vi "RemoteVI Launch Share.vi"(0 "VI":refnum<vi>, 1 "whole network?":bool, 2 "token":string, 3 "view only?":bool, 5 "port":u16=8088, 7 "fps":dbl=20.0, 8 "VI Server":string, 9 "window":u64, 10 "loop VI":path, 11 "error in":errorcluster) -> (4 "URL":string, 15 "error out":errorcluster)   [LabVIEW 2020, in "RemoteVI.lvlib"]
doc: "Starts one share (RemoteVI Start.vi and RemoteVI Start Window.vi call it): makes the access token (the given one or RemoteVI New Token.vi), the link (http://127.0.0.1:<port>/?t=... - or this computer's IP address with whole network?), refuses a port this application instance shares already (error 5001, RemoteVI Share Running.vi), opens a new clone of the reentrant RemoteVI Server Loop.vi, sets its controls and runs it (RemoteVI Launch Server Loop.vi), and waits until it listens (its listener error, e.g. 60; 5002 after 2 s). window not 0 shares that window of any process instead of VI (a window target). loop VI (not empty) runs that VI instead of the Server Loop (RemoteVI Start Landing Page.vi: the landing page)."
uses:
  RemoteVI.lvlib
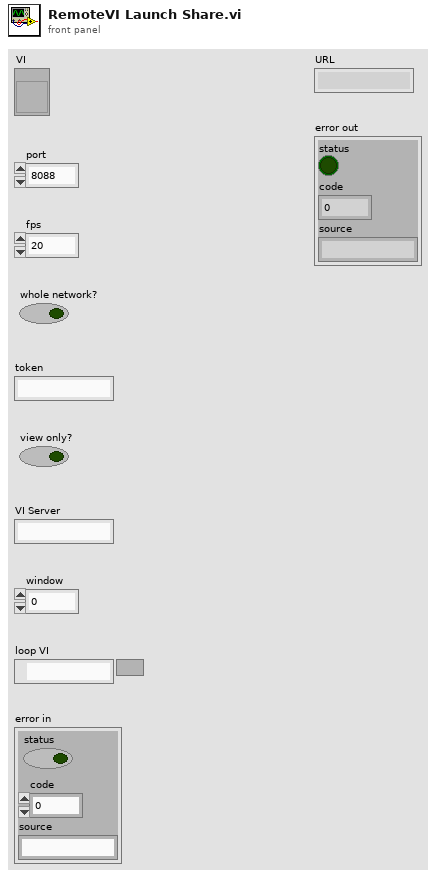
[diagram p1: front panel]
types:
  T1 = cluster{"token":string, "net address":u32, "url":string, "view only":bool, "whole network":bool, "window":u64}
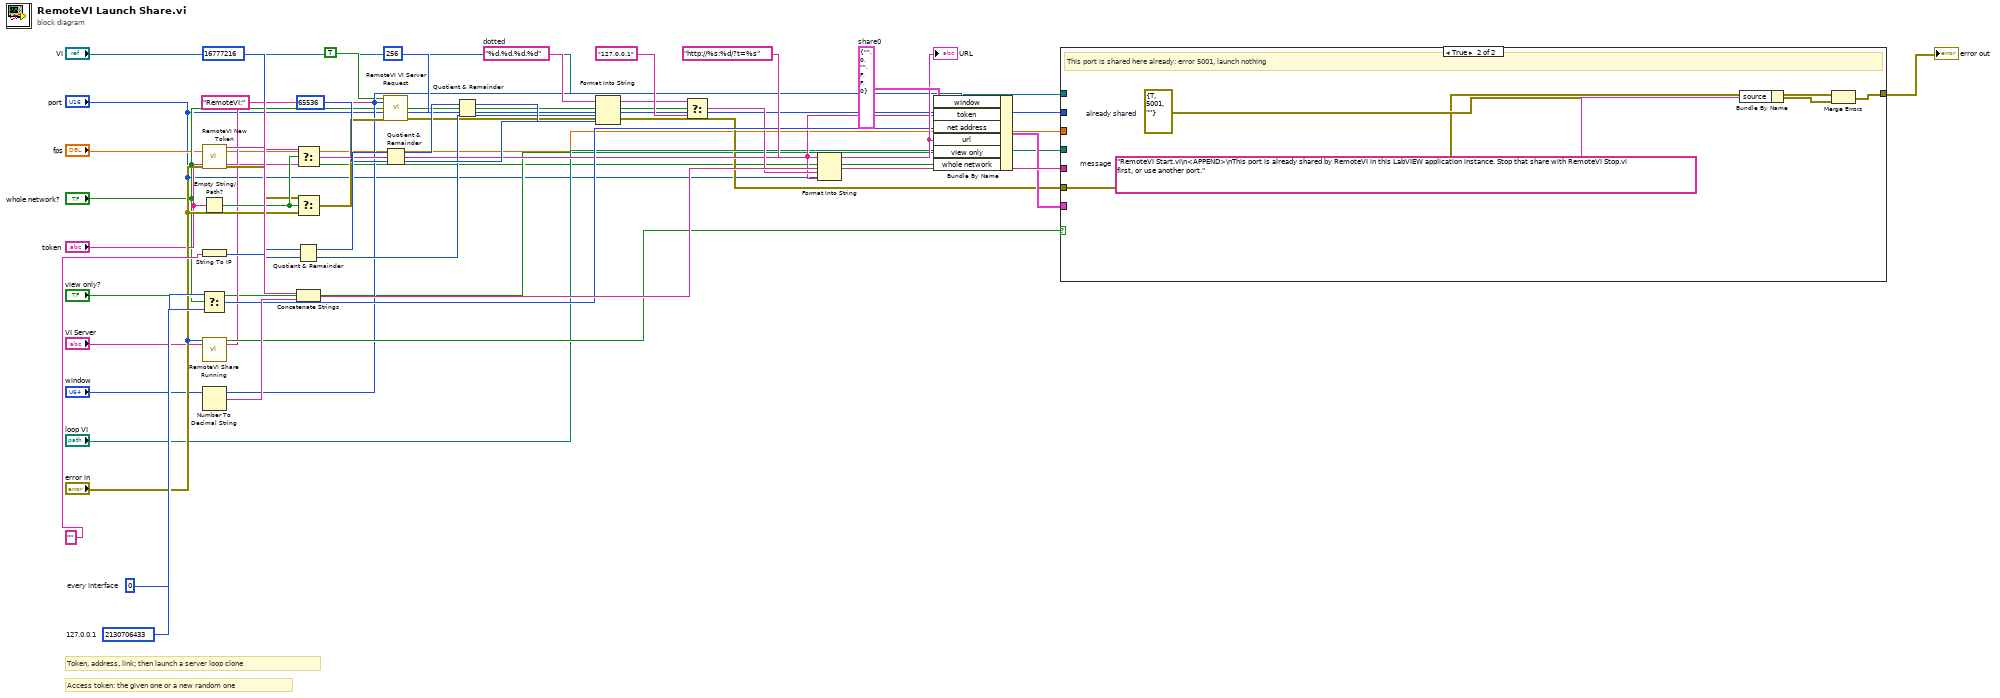
[diagram p0: block diagram]
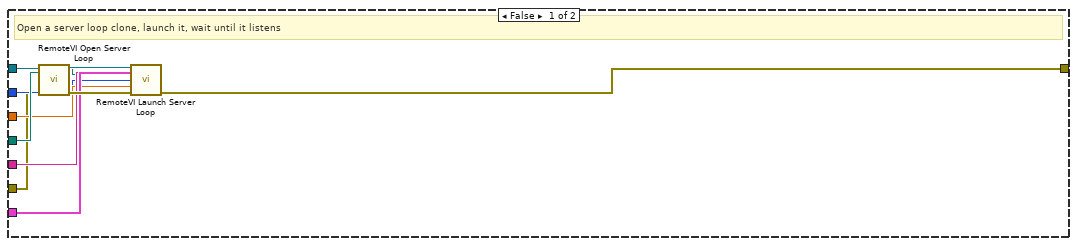
[diagram p2: hidden frame]
diagram:
  w38 = T1 {"token"="", "net address"=0, "url"="", "view only"=FALSE, "whole network"=FALSE, "window"=0}  # share0
  w34 = u32 2130706433  # 127.0.0.1
  w33 = u32 0  # every interface
  w29 = "%d.%d.%d.%d"  # dotted
  # "Access token: the given one or a new random one"
  # "Token, address, link; then launch a server loop clone"
  n1 = call "RemoteVI New Token.vi"("error in"="error in") -> ("token"=w14:string, "error out"=w15:errorcluster)  [unwired: 13 in]
  n2 = Empty String/Path?(string/path="token") -> (empty?=w16:bool)
  n3 = String To IP(1:"") -> (0:w19:u32)
  n4 = Select(t=w33, s="whole network?", f=w34) -> (s? t:f=w35:u32)
  n5 = call "RemoteVI Share Running.vi"("port"="port") -> ("running?"=w40:bool)  [unwired: 14 in]
  n6 = Number To Decimal String(number="port") -> (decimal integer string=w42:string)  [unwired: 1 in]
  n7 = Select(t=w14, s=w16, f="token") -> (s? t:f=w17:string)
  n8 = Select(t=w15, s=w16, f="error in") -> (s? t:f=w11:errorcluster)
  n9 = Quotient & Remainder(x=w19, y=u32 16777216) -> (x-y*floor(x/y)=w23:u32, floor(x/y)=w24:u32)
  n10 = Concatenate Strings("RemoteVI:", w42) -> (w43:string)
  n11 = call "RemoteVI VI Server Request.vi"("put?"=TRUE, "hWnd"="window", "address"="VI Server", "error in"=w11) -> ("error out"=w9:errorcluster)  [unwired: 9 in, 2 out]
  n12 = Quotient & Remainder(x=w23, y=u32 65536) -> (x-y*floor(x/y)=w25:u32, floor(x/y)=w26:u32)
  n13 = Quotient & Remainder(x=w25, y=u32 256) -> (x-y*floor(x/y)=w27:u32, floor(x/y)=w28:u32)
  n14 = Format Into String(format string=w29, w24, w26, w28, w27) -> (resulting string=w30:string)  [unwired: 2 in, 1 out]
  n15 = Select(t=w30, s="whole network?", f="127.0.0.1") -> (s? t:f=w32:string)
  n16 = Format Into String(format string="http://%s:%d/?t=%s", w32, "port", w17) -> (resulting string=w37:string)  [unwired: 2 in, 1 out]
  "URL" <- w37
  n17 = Bundle By Name(cluster=w38, "window"="window", "token"=w17, "net address"=w35, "url"=w37, "view only"="view only?", "whole network"="whole network?") -> (w39:T1)
  n18 = case shown="True" w40 {
    tunnel: "VI" -> [w46 _]
    tunnel: "port" -> [w47 _]
    tunnel: "fps" -> [w48 _]
    tunnel: "loop VI" -> [w51 _]
    tunnel: w43 -> [w49 _]
    tunnel: w9 -> [w45 w55]
    tunnel: [w54 w59] -> w44
    tunnel: w39 -> [w50 _]
    frame False {
      # "Open a server loop clone, launch it, wait until it listens"
      n19 = call "RemoteVI Open Server Loop.vi"("loop VI"=w51, "error in"=w45) -> ("Server Loop"=w52:refnum<vi>, "error out"=w53:errorcluster)  [unwired: 12 in]
      n20 = call "RemoteVI Launch Server Loop.vi"("Server Loop"=w52, "stop notifier name"=w49, "share"=w50, "VI"=w46, "port"=w47, "fps"=w48, "error in"=w53) -> ("error out"=w54:errorcluster)  [unwired: 8 in]
    }
    frame True {
      w57 = "RemoteVI Start.vi\n<APPEND>\nThis port is already shared by RemoteVI in this LabVIEW application instance. Stop that share with RemoteVI Stop.vi first, or use another port."  # message
      w56 = errorcluster {"status"=TRUE, "code"=5001, "source"=""}  # already shared
      # "This port is shared here already: error 5001, launch nothing"
      n21 = Bundle By Name(cluster=w56, "source"=w57) -> (w58:errorcluster)
      n22 = Merge Errors(w55, w58) -> (w59:errorcluster)
    }
  }
  "error out" <- w44
